vi "TMS Robot_adjust.vi"() -> ()   [LabVIEW 2018]
uses:
  <vilib>/Platform/TimedLoop/XDataNode/timing_clust.ctl
  <vilib>/Platform/TimedLoop/XDataNode/nitl_modes.ctl
  <vilib>/Platform/TimedLoop/XDataNode/wakeup.ctl
  <vilib>/myRIO/Instrument Drivers/Onboard IO/AI/typedefs/AI Reference.ctl
  <vilib>/myRIO/Common/Instrument Driver Framework/Utilities/typedefs/myRIO Generic Hardware Reference.ctl
  <vilib>/myRIO/Common/Instrument Driver Framework/Utilities/typedefs/Hardware Version Enum.ctl
  <vilib>/myRIO/Common/Instrument Driver Framework/Utilities/typedefs/myRIO v1.0 Reference.ctl
  <vilib>/myRIO/Common/Instrument Driver Framework/Utilities/typedefs/Generic FPGA Reference.ctl
  <vilib>/myRIO/Common/Instrument Driver Framework/myRIO v1.0/AI/typedefs/AI Channels List.ctl
  <vilib>/myRIO/Common/Instrument Driver Framework/myRIO v1.0/AI/typedefs/AI Channels Enum.ctl
  <vilib>/myRIO/Common/Instrument Driver Framework/Utilities/typedefs/Analog Scaling Constants List.ctl
  <vilib>/myRIO/Common/Instrument Driver Framework/Utilities/typedefs/Analog Scaling Constants.ctl
  <vilib>/userdefined/High Color/nirio_resource_hc.ctl
  <vilib>/myRIO/Instrument Drivers/Onboard IO/DIO/typedefs/DIO Reference.ctl
  <vilib>/myRIO/Common/Instrument Driver Framework/myRIO v1.0/DIO/typedefs/DIO Channels List.ctl
  <vilib>/myRIO/Common/Instrument Driver Framework/myRIO v1.0/DIO/typedefs/DIO Channels Enum.ctl
  <vilib>/myRIO/Common/Instrument Driver Framework/myRIO v1.0/AI/vis/myRIO v1.1 Open AI.vi
  <vilib>/myRIO/Common/Instrument Driver Framework/myRIO v1.0/DIO/vis/myRIO v1.1 Open DIO.vi
  <vilib>/myRIO/Common/Instrument Driver Framework/Utilities/vis/Validate Channels.vi
  <vilib>/myRIO/Common/Instrument Driver Framework/myRIO v1.0/AI/vis/myRIO v1.0 Reserve AI.vi
  <vilib>/myRIO/Common/Instrument Driver Framework/myRIO v1.0/DIO/vis/myRIO v1.0 Reserve DIO.vi
  <vilib>/myRIO/Common/Instrument Driver Framework/myRIO v1.0/DIO/vis/myRIO v1.0 Close DIO.vi
  <vilib>/myRIO/Common/Instrument Driver Framework/myRIO v1.0/AI/vis/myRIO v1.0 Build MUX Configuration AI.vi
  <vilib>/myRIO/Common/Instrument Driver Framework/myRIO v1.0/Resource Manager/vis/myRIO v1.0 Reserve Channel List.vi
  <vilib>/myRIO/Common/Instrument Driver Framework/myRIO v1.0/DIO/vis/myRIO v1.0 Build MUX Configuration DIO.vi
  <vilib>/myRIO/Common/Instrument Driver Framework/myRIO v1.0/DIO/vis/myRIO v1.0 Unreserve DIO.vi
  <vilib>/myRIO/Common/Instrument Driver Framework/myRIO v1.0/Resource Manager/vis/myRIO v1.0 Reserve Channel.vi
  <vilib>/myRIO/Common/Instrument Driver Framework/myRIO v1.0/Resource Manager/vis/myRIO v1.0 Unreserve Channel.vi
  <vilib>/myRIO/Common/Instrument Driver Framework/myRIO v1.0/Resource Manager/vis/myRIO v1.0 Create Configuration List.vi
  <vilib>/myRIO/Common/Instrument Driver Framework/myRIO v1.0/Resource Manager/vis/myRIO v1.0 Unreserve Channel List.vi
  <vilib>/myRIO/Common/Instrument Driver Framework/myRIO v1.0/Resource Manager/vis/myRIO v1.0 Build Mutex Name.vi
  <vilib>/Utility/VariantDataType/GetNumericInfo.vi
  <vilib>/Utility/error.llb/Error Cluster From Error Code.vi
  <vilib>/myRIO/Common/Instrument Driver Framework/myRIO v1.0/myRIO v1.1 Open.vi
  <vilib>/myRIO/Common/Instrument Driver Framework/Utilities/vis/IO Manager.vi
  <vilib>/myRIO/Common/Instrument Driver Framework/Utilities/vis/Configuration Manager.vi
  <vilib>/myRIO/Common/Instrument Driver Framework/myRIO v1.0/Resource Manager/vis/myRIO v1.0 Configure IO.vi
  <vilib>/myRIO/Common/Instrument Driver Framework/myRIO v1.0/myRIO v1.0 Close.vi
  <vilib>/myRIO/Common/Instrument Driver Framework/myRIO v1.0/AI/vis/myRIO v1.0 Get Scaling Constants AI.vi
  <vilib>/myRIO/Common/Instrument Driver Framework/myRIO v1.0/AI/vis/myRIO v1.0 Read AI.vi
  <vilib>/myRIO/Common/Instrument Driver Framework/myRIO v1.0/DIO/vis/myRIO v1.0 Write DIO.vi
  <vilib>/myRIO/Common/Instrument Driver Framework/myRIO v1.0/DIO/vis/myRIO v1.0 Shutdown DIO.vi
  <vilib>/platform/TimedLoop/XDataNode/XDataNode.xnode
  <vilib>/myRIO/Instrument Drivers/Onboard IO/DIO/vis/myRIO DIO Open.xnode
  <vilib>/myRIO/Instrument Drivers/Onboard IO/AI/vis/myRIO AI Open.xnode
  <vilib>/Platform/TimedLoop/XDataNode/XDNodeRunTimeDep.lvlib
  <vilib>/myRIO/Instrument Drivers/Onboard IO/DIO/DIO.lvlib
  <vilib>/myRIO/Instrument Drivers/Onboard IO/AI/AI.lvlib
panel:
  out "Optical R":dbl
  out "Optical L":dbl
  out "Optical psi":dbl
  out "Optical Z":dbl
  out "Optical Y":dbl
  out "Optical X":dbl
  in  "Stop number L":dbl
  in  "Stop number R":dbl
  in  "Stop number x":dbl
  in  "Stop number y":dbl
  in  "Stop number z":dbl
  in  "Stop number psi":dbl
  out "up L":bool
  out "left L":bool
  in  "Step/s  curve":dbl=4.0
  in  "Step difference L":dbl
  in  "Tab Control":enum32{"Azimuth", "Elevation"}(tab)
  in  "Right":bool
  in  "Left":bool
  out "Real Output theta":dbl
  in  "User Input theta":dbl
  in  "Up":bool
  in  "Down":bool
  out "Real Output Phi":dbl
  in  "User Input Phi":dbl=10.45218049
  in  "Motor Input L":dbl
  out "down L":bool
  out "right L":bool
  out "Moving":bool
  out "up R":bool
  out "left R":bool
  in  "Step difference R":dbl
  in  "Motor Input R":dbl
  out "down R":bool
  out "right R":bool
  out "Moving R":bool
  out "up z":bool
  out "down z":bool
  out "right z":bool
  out "left z":bool
  in  "Step/s z":dbl=4.0
  out "Motor Position z":dbl
  in  "User Input z":dbl
  out "Motor State z":dbl
  out "Real Output z":dbl
  in  "Step diff z":dbl
  in  "Up z":bool
  in  "Motor Input z":dbl
  in  "Down z":bool
  out "Moving z":bool
  out "up x":bool
  out "down x":bool
  out "right x":bool
  out "left x":bool
  in  "Step/s x":dbl=4.0
  out "Motor Position x":dbl
  in  "User Input x":dbl
  out "Motor State x":dbl
  out "Real Output x":dbl
  in  "Step diff x":dbl
  in  "Forward x":bool
  in  "Motor Input x":dbl
  in  "Backward x":bool
  out "Moving x":bool
  out "up y":bool
  out "down y":bool
  out "right y":bool
  out "left y":bool
  in  "Step/s y":dbl=4.0
  out "Motor Position y":dbl
  in  "User Input y":dbl
  out "Motor State y":dbl
  out "Real Output y":dbl
  in  "Step diff y":dbl
  in  "Left y":bool
  in  "Motor Input y":dbl
  in  "Right y":bool
  out "Moving y":bool
  out "up psi":bool
  out "down psi":bool
  out "right psi":bool
  out "left psi":bool
  in  "Step/s psi":dbl=4.0
  out "Motor Position psi":dbl
  in  "User Input psi":dbl
  out "Motor State psi":dbl
  out "Real Output psi":dbl
  in  "Step diff psi":dbl
  in  "Left psi":bool
  in  "Motor Input psi":dbl
  in  "Right psi":bool
  out "Moving psi":bool
  in  "Stop":bool
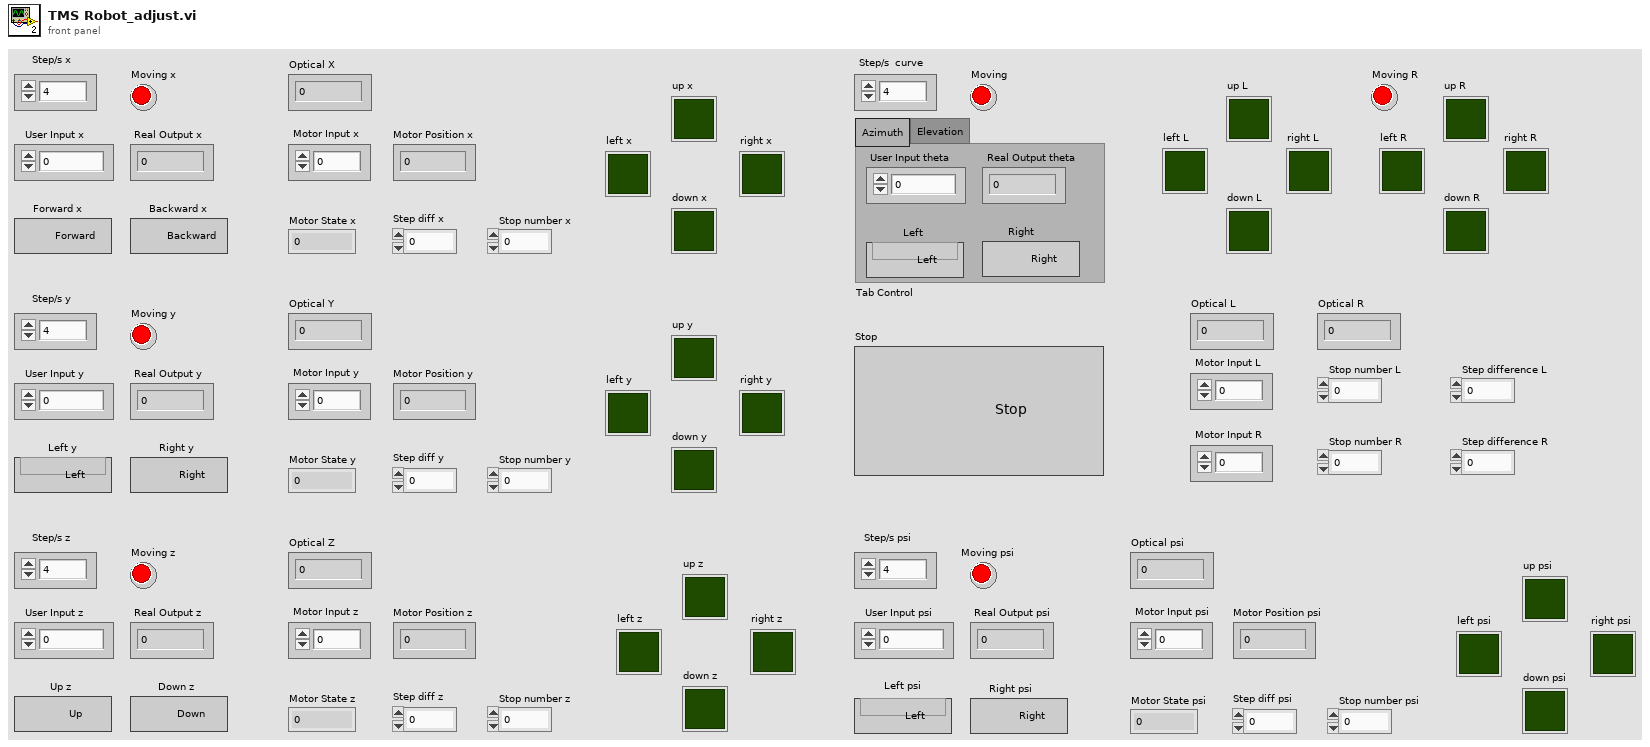
[diagram p1: front panel]
types:
  T1 = typedef "nirio_resource_hc.ctl" = tag
  T2 = typedef "Hardware Version Enum.ctl" = enum16{"Unknown", "myRIO-1900", "myRIO-1950", "roboRIO", "NI ELVIS RIO CM", "ELVIS III"}
  T3 = typedef "XDNodeRunTimeDep.lvlib/timing_clust.ctl" = cluster{"Expected End [f-1]":u64, "Actual End [f-1]":u64, "Finished Late? [f-1]":bool, "Expected End [i-1]":u64, "Actual End [i-1]":u64, "Finished Late? [i-1]":bool, "Expected Start [i]":u64, "Actual Start [i]":u64, "Expected Start [f]":u64, "Actual Start [f]":u64, "Source Name":string, "Structure Name":string, "Period":i64, "Deadline":i64, "Offset":i64, "Start":i64, "Priority":i32, "Timeout":i32, "Mode":T4, "Wakeup Reason":T5, "Error":errorcluster, "Source Type":string, "Secondary Source Type":string, "Global End Time":u64, "Global Start Time":u64, "Frame Duration":u64, "Iteration Duration":u64, "Assigned CPU":i32, "I/O Scan Engine Mode":u32}
  T4 = typedef "XDNodeRunTimeDep.lvlib/nitl_modes.ctl" = enum32{"No Change", "Process missed periods, maintain original phase", "Discard missed periods, maintain original phase", "Process missed periods, ignore original phase", "Discard missed periods, ignore original phase"}
  T5 = typedef "XDNodeRunTimeDep.lvlib/wakeup.ctl" = enum32{"Normal", "Aborted", "Asynchronous wakeup", "Timing source error", "Timed loop error", "Timeout"}
  T6 = typedef "AI.lvlib/AI Reference.ctl" = cluster{"myRIO Reference":T7, "AI Channels List":T10, "AI Scaling Constants List":T12}
  T7 = typedef "myRIO Generic Hardware Reference.ctl" = cluster{"myRIO Model":T2, "myRIO Hardware Reference":T8}
  T8 = typedef "myRIO v1.0 Reference.ctl" = cluster{"Generic FPGA Reference":T9, "Allow multiple opens":bool}
  T9 = typedef "Generic FPGA Reference.ctl" = refnum<k20>
  T10 = typedef "AI Channels List.ctl" = T11[]
  T11 = typedef "AI Channels Enum.ctl" = enum16{"Not Connected", "AudioIn/Left", "AudioIn/Right", "C/AI0", "C/AI1", "A/AI0", "A/AI1", "A/AI2", "A/AI3", "A/AI4", "A/AI5", "A/AI6", "A/AI7", "B/AI0", "B/AI1", "B/AI2", "B/AI3", "B/AI4", "B/AI5", "B/AI6", "B/AI7", "AI/AI0", "AI/AI1", "AI/AI2", "AI/AI3", "A/AI0 (DIFF)", "A/AI1 (DIFF)", "A/AI2 (DIFF)", "A/AI3 (DIFF)", "B/AI0 (DIFF)", "B/AI1 (DIFF)", "B/AI2 (DIFF)", "B/AI3 (DIFF)"}
  T12 = typedef "Analog Scaling Constants List.ctl" = T13[]
  T13 = typedef "Analog Scaling Constants.ctl" = cluster{"LSB Weight (Volts)":dbl, "Offset (Volts)":dbl, "Signed?":bool}
  T14 = typedef "DIO.lvlib/DIO Reference.ctl" = cluster{"myRIO Reference":T7, "DIO Channels List":T15}
  T15 = typedef "DIO Channels List.ctl" = T16[]
  T16 = typedef "DIO Channels Enum.ctl" = enum16{"Not Connected", "C/DIO0", "C/DIO1", "C/DIO2", "C/DIO3", "C/DIO4", "C/DIO5", "C/DIO6", "C/DIO7", "A/DIO0", "A/DIO1", "A/DIO2", "A/DIO3", "A/DIO4", "A/DIO5", "A/DIO6", "A/DIO7", "A/DIO8", "A/DIO9", "A/DIO10", "A/DIO11", "A/DIO12", "A/DIO13", "A/DIO14", "A/DIO15", "A/DIO16", "A/DIO17", "A/DIO18", "A/DIO19", "B/DIO0", "B/DIO1", "B/DIO2", "B/DIO3", "B/DIO4", "B/DIO5", "B/DIO6", "B/DIO7", "B/DIO8", "B/DIO9", "B/DIO10", "B/DIO11", "B/DIO12", "B/DIO13", "B/DIO14", "B/DIO15", "B/DIO16", "B/DIO17", "B/DIO18", "B/DIO19", "LED0", "LED1", "LED2", "LED3", "Button0", "DIO/DIO0", "DIO/DIO1", "DIO/DIO2", "DIO/DIO3", "DIO/DIO4", "DIO/DIO5", "DIO/DIO6", "DIO/DIO7", "DIO/DIO8", "DIO/DIO9", "SPI/CS0", "SPI/CS1", "SPI/CS2", "SPI/CS3", "LED RADIO (Green)", "LED RADIO (Red)", "LED COMM (Green)", "LED COMM (Red)", "LED MODE (Green)", "LED MODE (Red)"}
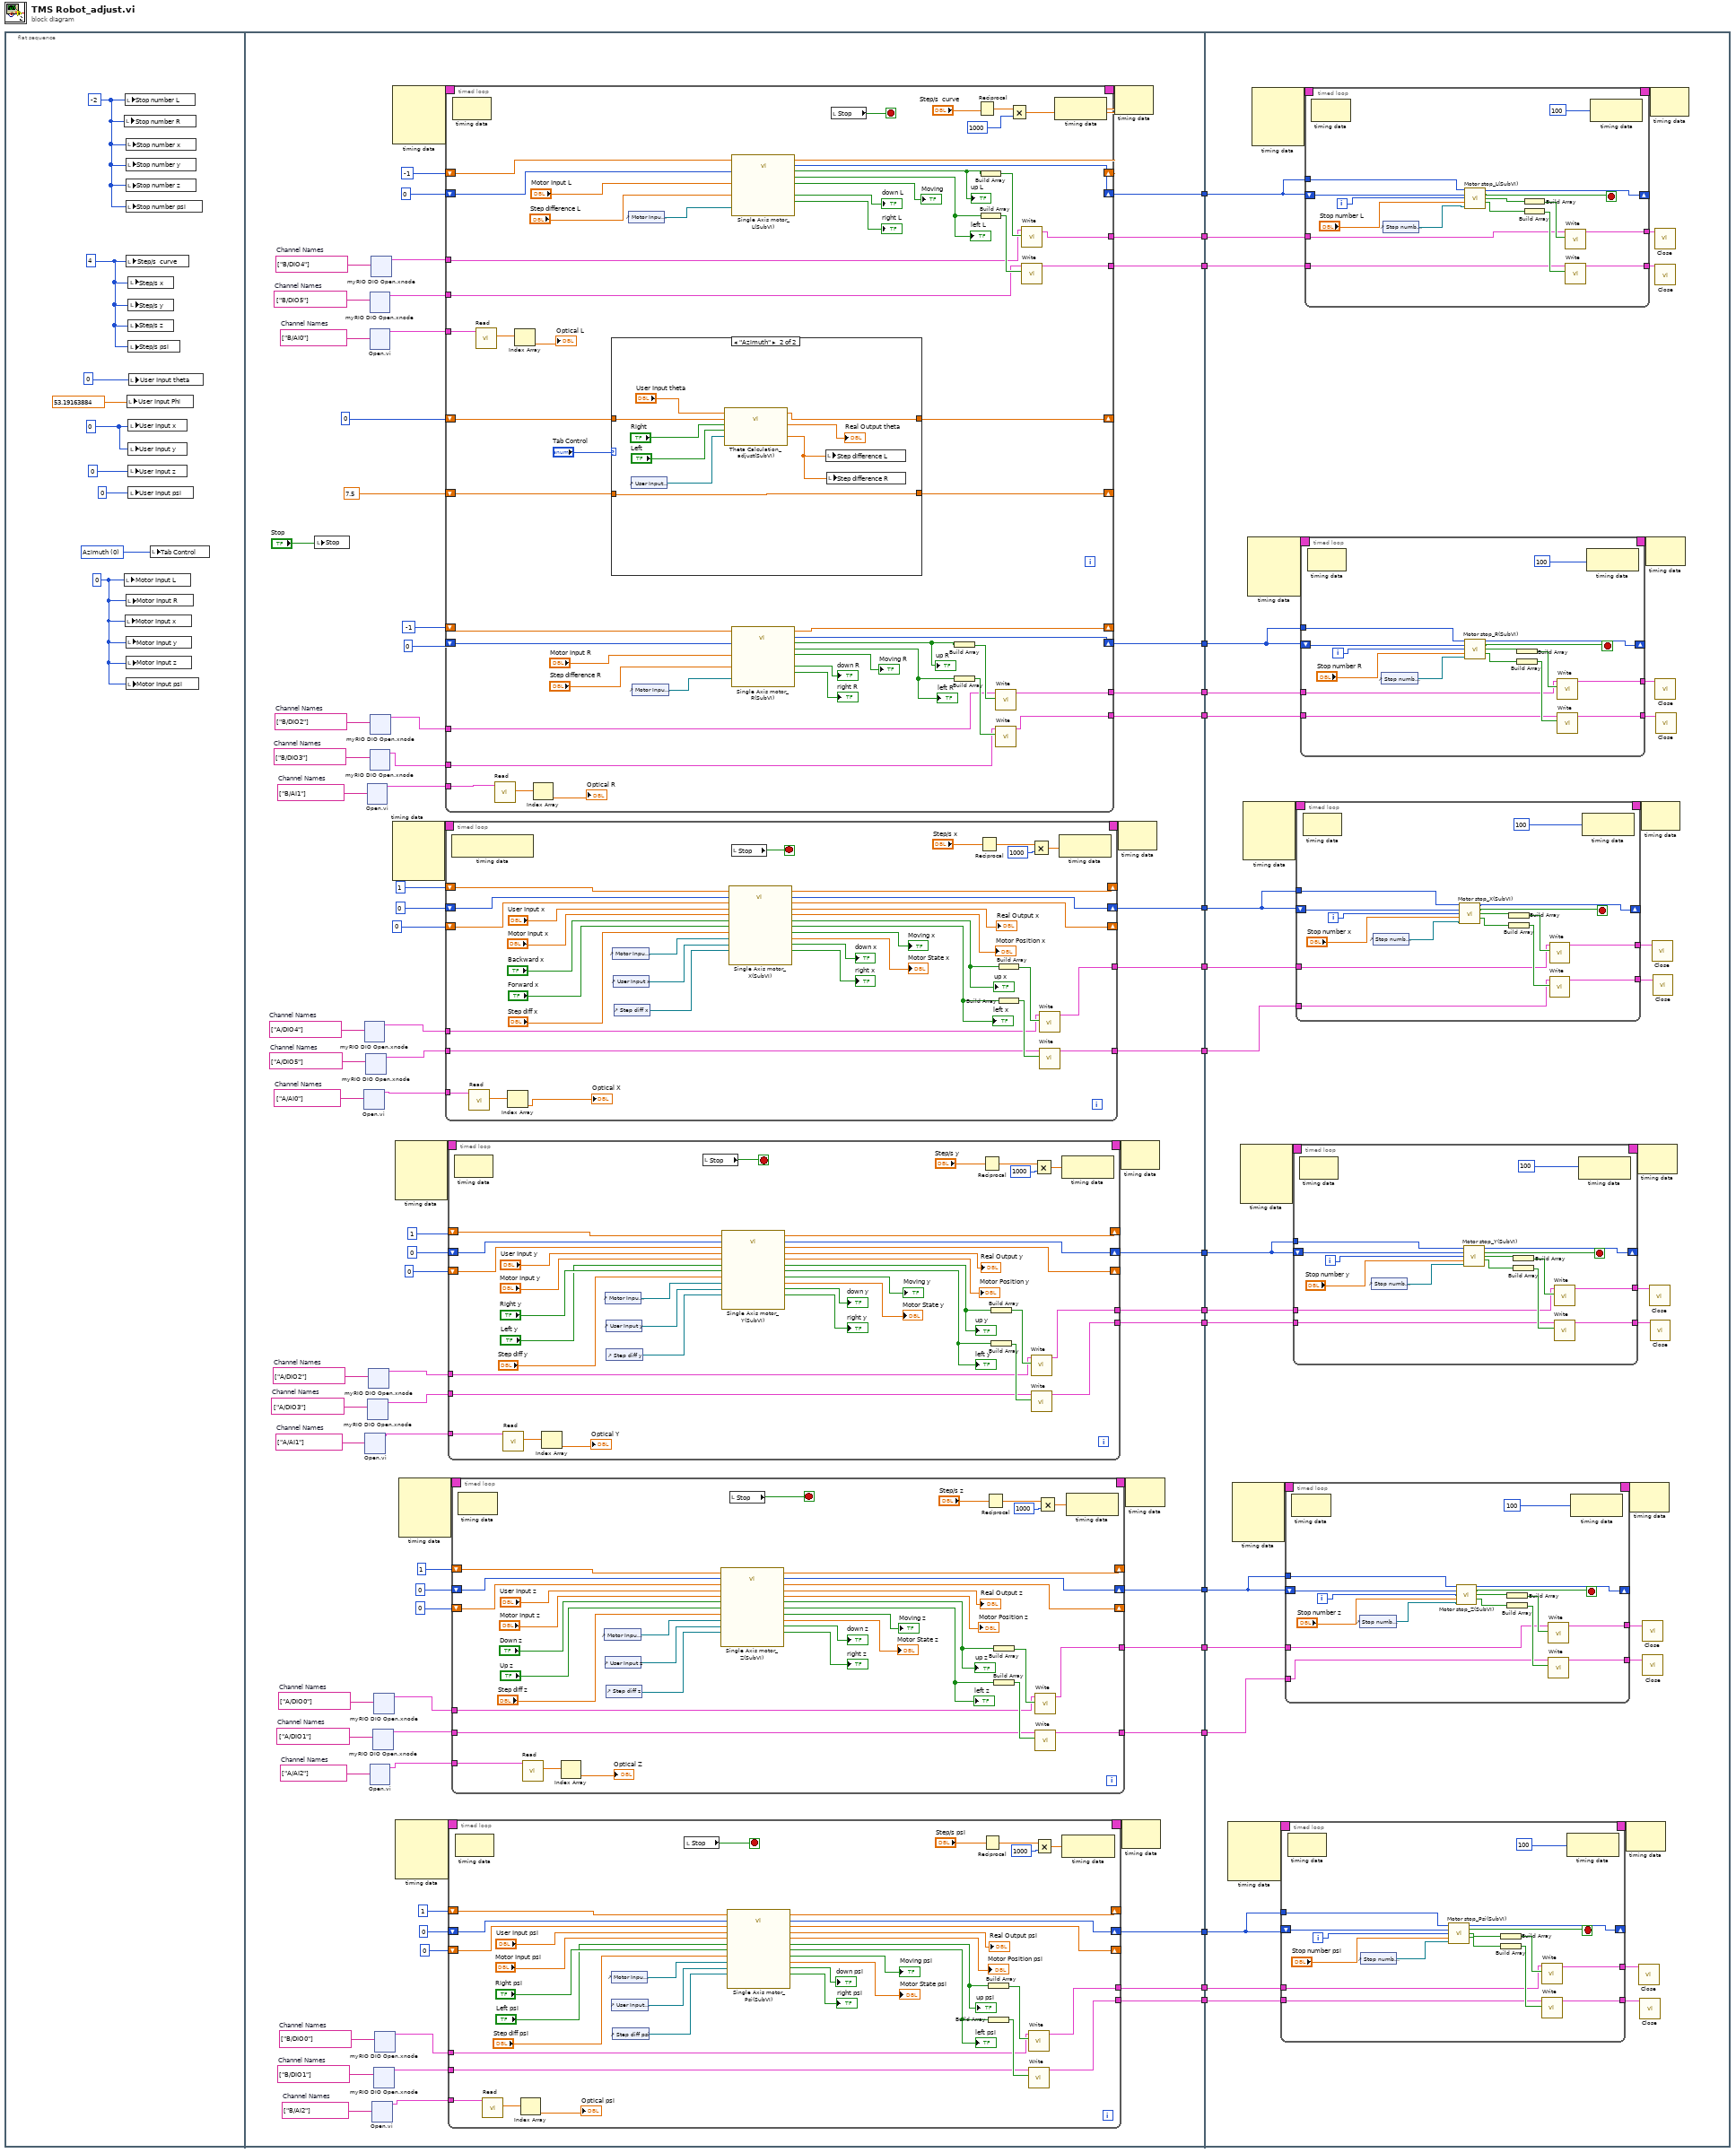
[diagram p0: block diagram]
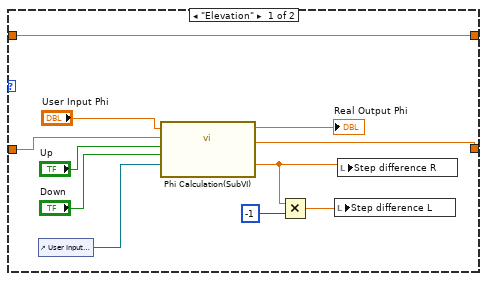
[diagram p2: hidden frame]
diagram:
  n1 = flat-sequence {
    tunnel: [w88] -> w18
    tunnel: [w87] -> w17
    tunnel: [w86] -> w16
    tunnel: [w85] -> w15
    tunnel: [w84] -> w14
    tunnel: [w83] -> w13
    tunnel: [w82] -> w12
    tunnel: [w81] -> w11
    tunnel: [w80] -> w10
    tunnel: [w79] -> w9
    tunnel: [w78] -> w8
    tunnel: [w77] -> w7
    tunnel: [w76] -> w6
    tunnel: [w75] -> w5
    tunnel: [w74] -> w4
    tunnel: [w73] -> w3
    tunnel: [w72] -> w2
    tunnel: [w71] -> w1
    tunnel: w18 -> [w696]
    tunnel: w17 -> [w693]
    tunnel: w16 -> [w690]
    tunnel: w15 -> [w687]
    tunnel: w14 -> [w684]
    tunnel: w13 -> [w681]
    tunnel: w12 -> [w678]
    tunnel: w11 -> [w677]
    tunnel: w10 -> [w676]
    tunnel: w9 -> [w675]
    tunnel: w8 -> [w670]
    tunnel: w7 -> [w669]
    tunnel: w6 -> [w668]
    tunnel: w5 -> [w667]
    tunnel: w4 -> [w666]
    tunnel: w3 -> [w665]
    tunnel: w2 -> [w664]
    tunnel: w1 -> [w663]
    frame #0 {
      w19 = 0
      w20 = u16 0 items=["Azimuth"]
      w22 = 0
      w26 = -2
      w25 = 4
      n2 = local write "Stop number R"(w26) -> ()
      n3 = local write "Motor Input L"(w19) -> ()
      n4 = local write "Stop number L"(w26) -> ()
      n5 = local write "Motor Input x"(w19) -> ()
      n6 = local write "Stop number x"(w26) -> ()
      n7 = local write "Stop number y"(w26) -> ()
      n8 = local write "Stop number z"(w26) -> ()
      n9 = local write "Stop number psi"(w26) -> ()
      n10 = local write "Motor Input R"(w19) -> ()
      n11 = local write "Motor Input y"(w19) -> ()
      n12 = local write "Motor Input z"(w19) -> ()
      n13 = local write "Motor Input psi"(w19) -> ()
      n14 = local write "Step/s  curve"(w25) -> ()
      n15 = local write "User Input Phi"(53.19163884) -> ()
      n16 = local write "Step/s x"(w25) -> ()
      n17 = local write "Step/s y"(w25) -> ()
      n18 = local write "Step/s z"(w25) -> ()
      n19 = local write "Step/s psi"(w25) -> ()
      n20 = local write "User Input x"(w22) -> ()
      n21 = local write "User Input y"(w22) -> ()
      n22 = local write "User Input z"(0) -> ()
      n23 = local write "User Input psi"(0) -> ()
      n24 = local write "User Input theta"(0) -> ()
      n25 = local write "Tab Control"(w20) -> ()
    }
    frame #1 {
      w36 = tag[] ["B/AI0"]  # Channel Names
      w38 = tag[] ["B/AI1"]  # Channel Names
      w41 = tag[] ["B/AI2"]  # Channel Names
      w43 = tag[] ["A/AI2"]  # Channel Names
      w45 = tag[] ["A/AI1"]  # Channel Names
      w47 = tag[] ["A/AI0"]  # Channel Names
      w51 = tag[] ["B/DIO1"]  # Channel Names
      w50 = tag[] ["B/DIO0"]  # Channel Names
      w55 = tag[] ["A/DIO1"]  # Channel Names
      w54 = tag[] ["A/DIO0"]  # Channel Names
      w59 = tag[] ["A/DIO3"]  # Channel Names
      w58 = tag[] ["A/DIO2"]  # Channel Names
      w63 = tag[] ["A/DIO5"]  # Channel Names
      w62 = tag[] ["A/DIO4"]  # Channel Names
      w67 = tag[] ["B/DIO5"]  # Channel Names
      w66 = tag[] ["B/DIO4"]  # Channel Names
      w70 = tag[] ["B/DIO3"]  # Channel Names
      w69 = tag[] ["B/DIO2"]  # Channel Names
      n26 = local write "Stop"("Stop") -> ()
      n27 = xnode "Open.vi"("Channel Names"=w47) -> ("AI Ref Out"=w46:T6)  [unwired: 2 in, 1 out]
      n28 = xnode "myRIO DIO Open.xnode"("Channel Names"=w62) -> ("DIO Ref Out"=w61:T14)  [unwired: 2 in, 1 out]
      n29 = xnode "Open.vi"("Channel Names"=w45) -> ("AI Ref Out"=w44:T6)  [unwired: 2 in, 1 out]
      n30 = xnode "myRIO DIO Open.xnode"("Channel Names"=w63) -> ("DIO Ref Out"=w60:T14)  [unwired: 2 in, 1 out]
      n31 = xnode "Open.vi"("Channel Names"=w38) -> ("AI Ref Out"=w37:T6)  [unwired: 2 in, 1 out]
      n32 = xnode "myRIO DIO Open.xnode"("Channel Names"=w59) -> ("DIO Ref Out"=w56:T14)  [unwired: 2 in, 1 out]
      n33 = xnode "myRIO DIO Open.xnode"("Channel Names"=w58) -> ("DIO Ref Out"=w57:T14)  [unwired: 2 in, 1 out]
      n34 = xnode "myRIO DIO Open.xnode"("Channel Names"=w67) -> ("DIO Ref Out"=w64:T14)  [unwired: 2 in, 1 out]
      n35 = xnode "Open.vi"("Channel Names"=w36) -> ("AI Ref Out"=w35:T6)  [unwired: 2 in, 1 out]
      n36 = xnode "myRIO DIO Open.xnode"("Channel Names"=w70) -> ("DIO Ref Out"=w39:T14)  [unwired: 2 in, 1 out]
      n37 = xnode "Open.vi"("Channel Names"=w43) -> ("AI Ref Out"=w42:T6)  [unwired: 2 in, 1 out]
      n38 = xnode "myRIO DIO Open.xnode"("Channel Names"=w69) -> ("DIO Ref Out"=w68:T14)  [unwired: 2 in, 1 out]
      n39 = xnode "myRIO DIO Open.xnode"("Channel Names"=w66) -> ("DIO Ref Out"=w65:T14)  [unwired: 2 in, 1 out]
      n40 = xnode "Open.vi"("Channel Names"=w41) -> ("AI Ref Out"=w40:T6)  [unwired: 2 in, 1 out]
      n41 = xnode "myRIO DIO Open.xnode"("Channel Names"=w55) -> ("DIO Ref Out"=w52:T14)  [unwired: 2 in, 1 out]
      n42 = xnode "myRIO DIO Open.xnode"("Channel Names"=w54) -> ("DIO Ref Out"=w53:T14)  [unwired: 2 in, 1 out]
      n43 = xnode "myRIO DIO Open.xnode"("Channel Names"=w51) -> ("DIO Ref Out"=w48:T14)  [unwired: 2 in, 1 out]
      n44 = xnode "myRIO DIO Open.xnode"("Channel Names"=w50) -> ("DIO Ref Out"=w49:T14)  [unwired: 2 in, 1 out]
      n45 = node-c288() -> (w103:T3)  [unwired: 4 in]
      n46 = node-c288() -> (w110:T3)  [unwired: 4 in]
      n47 = node-c288() -> (w101:T3)  [unwired: 4 in]
      n48 = node-c288() -> (w93:T3)  [unwired: 4 in]
      n49 = node-c288() -> (w105:T3)  [unwired: 4 in]
      n50 = timed-loop {
        shift-right: [w514] -> w86
        shift-left: 0 -> [w525]
        shift-right: [w515] -> _
        shift-left: 1 -> [w526]
        shift-right: [w510] -> _
        shift-left: 0 -> [w524]
        timing: w103 -> [_]
        timing-out: [_] -> w102
        tunnel: w61 -> [w501]
        tunnel: w60 -> [w500]
        tunnel: [w499] -> w78
        tunnel: [w498] -> w77
        tunnel: w46 -> [w496]
        stop <- w508 stop-if-true
        n51 = node-c288() -> ()  [unwired: 1 in, 1 out]
        n52 = call <vilib>:"Read.vi"("AI Ref In"=w496) -> ("Values"=w497:dbl[])  [unwired: 8 in, 2 out]
        n53 = Index Array(array=w497) -> (element=→"Optical X":dbl)  [unwired: 1 in]
        n54 = control-ref of="Motor Input x"() -> (w518:refnum<vi>)
        n55 = control-ref of="User Input x"() -> (w517:refnum<vi>)
        n56 = control-ref of="Step diff x"() -> (w516:refnum<vi>)
        n57 = call "Single Axis motor_X(SubVI).vi"("State=1, I"=w526, "Motor=0, I"=w525, "Position=0, I"=w524, "User Input"="User Input x", "Motor Input"="Motor Input x", "Backward"="Backward x", "Forward"="Forward x", "Step diff"="Step diff x", "Motor input_L"=w518, "User input_L"=w517, "Step diff_L"=w516) -> ("right"=→"right x":bool, "down"=→"down x":bool, "Motor State"=→"Motor State x":dbl, "State=1, O"=w515:dbl, "Motor=0, O"=w514:i32, "Position=0, O"=w510:dbl, "Real Output"=→"Real Output x":dbl, "Motor Position"=→"Motor Position x":dbl, "up"=w503:bool, "left"=w502:bool, "Moving"=→"Moving x":bool)  [unwired: 5 in, 1 out]
        "up x" <- w503
        "left x" <- w502
        n58 = local read "Stop"() -> (w508:bool)
        n59 = Reciprocal(x="Step/s x") -> (1/x=w529:dbl)
        n60 = Build Array(w503) -> (w505:bool[])
        n61 = Build Array(w502) -> (w504:bool[])
        n62 = Multiply(x=w529, y=1000) -> (x*y=w527:dbl)
        n63 = call <vilib>:"Write.vi"("Values"=w505, "DIO Ref In"=w501) -> ("DIO Ref Out"=w498:T14)  [unwired: 7 in, 1 out]
        n64 = call <vilib>:"Write.vi"("Values"=w504, "DIO Ref In"=w500) -> ("DIO Ref Out"=w499:T14)  [unwired: 7 in, 1 out]
        n65 = node-c288(w527) -> ()  [unwired: 1 out]
      }
      n66 = timed-loop {
        shift-right: [w618] -> w88
        shift-left: 0 -> [w619]
        shift-right: [w620] -> _
        shift-left: -1 -> [w621]
        shift-right: [w625] -> _
        shift-left: 0 -> [w626]
        timing: w110 -> [_]
        timing-out: [_] -> w109
        shift-right: [w623] -> _
        shift-left: 7.5 -> [w622]
        shift-right: [w607] -> w87
        shift-left: 0 -> [w608]
        shift-right: [w605] -> _
        shift-left: -1 -> [w606]
        tunnel: w68 -> [w596]
        tunnel: w39 -> [w595]
        tunnel: w64 -> [w590]
        tunnel: w65 -> [w589]
        tunnel: [w588] -> w82
        tunnel: [w587] -> w81
        tunnel: [w586] -> w80
        tunnel: [w585] -> w79
        tunnel: w37 -> [w583]
        tunnel: w35 -> [w581]
        stop <- w613 stop-if-true
        n67 = node-c288() -> ()  [unwired: 1 in, 1 out]
        n68 = call <vilib>:"Read.vi"("AI Ref In"=w581) -> ("Values"=w582:dbl[])  [unwired: 8 in, 2 out]
        n69 = call <vilib>:"Read.vi"("AI Ref In"=w583) -> ("Values"=w584:dbl[])  [unwired: 8 in, 2 out]
        n70 = Index Array(array=w582) -> (element=→"Optical L":dbl)  [unwired: 1 in]
        n71 = Index Array(array=w584) -> (element=→"Optical R":dbl)  [unwired: 1 in]
        n72 = case shown="\"Azimuth\"" "Tab Control" {
          tunnel: w622 -> [w640 w650]
          tunnel: [w639 w650] -> w623
          tunnel: w626 -> [w641 w647]
          tunnel: [w641 w646] -> w625
          frame "Elevation" {
            n73 = control-ref of="User Input Phi"() -> (w634:refnum<vi>)
            n74 = call "Phi Calculation(SubVI).vi"(0:"User Input Phi"="User Input Phi", "Position=0, I"=w640, "Up"="Up", "Down"="Down", 11:"User Input Phi"=w634) -> ("Real output phi"=→"Real Output Phi":dbl, "Position=0, O"=w639:dbl, "Step diff"=w631:dbl)  [unwired: 8 in]
            n75 = Multiply(x=w631, y=-1) -> (x*y=w632:dbl)
            n76 = local write "Step difference L"(w632) -> ()
            n77 = local write "Step difference R"(w631) -> ()
          }
          frame "Azimuth" {
            n78 = control-ref of="User Input theta"() -> (w648:refnum<vi>)
            n79 = call "Theta Calculation_adjust(SubVI).vi"(0:"User Input theta"="User Input theta", "Position=-85, I"=w647, "Right"="Right", "Left"="Left", 11:"User Input theta"=w648) -> ("Position=-85, O"=w646:dbl, "Real output theta"=→"Real Output theta":dbl, "Step diff"=w644:dbl)  [unwired: 8 in]
            n80 = local write "Step difference L"(w644) -> ()
            n81 = local write "Step difference R"(w644) -> ()
          }
        }
        n82 = control-ref of="Motor Input L"() -> (w615:refnum<vi>)
        n83 = control-ref of="Motor Input R"() -> (w610:refnum<vi>)
        n84 = call "Single Axis motor_R(SubVI).vi"("State=1, I"=w606, "Motor=0, I"=w608, "Motor Input"="Motor Input R", "Step diff"="Step difference R", "Motor Input_L"=w610) -> ("right"=→"right R":bool, "State=1, O"=w605:dbl, "Motor=0, O"=w607:i32, "up"=w598:bool, "left"=w597:bool, "Moving"=→"Moving R":bool, "down"=→"down R":bool)  [unwired: 14 in, 2 out]
        "up R" <- w598
        "left R" <- w597
        n85 = call "Single Axis motor_L(SubVI).vi"("State=1, I"=w621, "Motor=0, I"=w619, "Motor Input"="Motor Input L", "Step diff"="Step difference L", "Motor Input_L"=w615) -> ("right"=→"right L":bool, "State=1, O"=w620:dbl, "Motor=0, O"=w618:i32, "up"=w592:bool, "left"=w591:bool, "Moving"=→"Moving":bool, "down"=→"down L":bool)  [unwired: 14 in, 2 out]
        "up L" <- w592
        "left L" <- w591
        n86 = local read "Stop"() -> (w613:bool)
        n87 = Build Array(w598) -> (w600:bool[])
        n88 = Build Array(w597) -> (w599:bool[])
        n89 = Reciprocal(x="Step/s  curve") -> (1/x=w629:dbl)
        n90 = Build Array(w592) -> (w594:bool[])
        n91 = Build Array(w591) -> (w593:bool[])
        n92 = call <vilib>:"Write.vi"("Values"=w600, "DIO Ref In"=w596) -> ("DIO Ref Out"=w586:T14)  [unwired: 7 in, 1 out]
        n93 = call <vilib>:"Write.vi"("Values"=w599, "DIO Ref In"=w595) -> ("DIO Ref Out"=w585:T14)  [unwired: 7 in, 1 out]
        n94 = Multiply(x=w629, y=1000) -> (x*y=w627:dbl)
        n95 = call <vilib>:"Write.vi"("Values"=w594, "DIO Ref In"=w589) -> ("DIO Ref Out"=w588:T14)  [unwired: 7 in, 1 out]
        n96 = call <vilib>:"Write.vi"("Values"=w593, "DIO Ref In"=w590) -> ("DIO Ref Out"=w587:T14)  [unwired: 7 in, 1 out]
        n97 = node-c288(w627) -> ()  [unwired: 1 out]
      }
      n98 = timed-loop {
        shift-right: [w472] -> w85
        shift-left: 0 -> [w483]
        shift-right: [w473] -> _
        shift-left: 1 -> [w484]
        shift-right: [w469] -> _
        shift-left: 0 -> [w482]
        timing: w101 -> [_]
        timing-out: [_] -> w100
        tunnel: w57 -> [w459]
        tunnel: w56 -> [w458]
        tunnel: [w457] -> w76
        tunnel: [w456] -> w75
        tunnel: w44 -> [w454]
        stop <- w467 stop-if-true
        n99 = node-c288() -> ()  [unwired: 1 in, 1 out]
        n100 = call <vilib>:"Read.vi"("AI Ref In"=w454) -> ("Values"=w455:dbl[])  [unwired: 8 in, 2 out]
        n101 = Index Array(array=w455) -> (element=→"Optical Y":dbl)  [unwired: 1 in]
        n102 = control-ref of="Motor Input y"() -> (w476:refnum<vi>)
        n103 = control-ref of="User Input y"() -> (w475:refnum<vi>)
        n104 = control-ref of="Step diff y"() -> (w474:refnum<vi>)
        n105 = local read "Stop"() -> (w467:bool)
        n106 = call "Single Axis motor_Y(SubVI).vi"("State=1, I"=w484, "Motor=0, I"=w483, "Position=0, I"=w482, "User Input"="User Input y", "Motor Input"="Motor Input y", "Backward"="Left y", "Forward"="Right y", "Step diff"="Step diff y", "Motor input_L"=w476, "User input_L"=w475, "Step diff_L"=w474) -> ("right"=→"right y":bool, "down"=→"down y":bool, "Motor State"=→"Motor State y":dbl, "State=1, O"=w473:dbl, "Motor=0, O"=w472:i32, "Position=0, O"=w469:dbl, "Real Output"=→"Real Output y":dbl, "Motor Position"=→"Motor Position y":dbl, "up"=w461:bool, "left"=w460:bool, "Moving"=→"Moving y":bool)  [unwired: 5 in, 1 out]
        "up y" <- w461
        "left y" <- w460
        n107 = Reciprocal(x="Step/s y") -> (1/x=w487:dbl)
        n108 = Build Array(w461) -> (w463:bool[])
        n109 = Build Array(w460) -> (w462:bool[])
        n110 = call <vilib>:"Write.vi"("Values"=w463, "DIO Ref In"=w459) -> ("DIO Ref Out"=w456:T14)  [unwired: 7 in, 1 out]
        n111 = call <vilib>:"Write.vi"("Values"=w462, "DIO Ref In"=w458) -> ("DIO Ref Out"=w457:T14)  [unwired: 7 in, 1 out]
        n112 = Multiply(x=w487, y=1000) -> (x*y=w485:dbl)
        n113 = node-c288(w485) -> ()  [unwired: 1 out]
      }
      n114 = timed-loop {
        shift-right: [w430] -> w83
        shift-left: 0 -> [w441]
        shift-right: [w431] -> _
        shift-left: 1 -> [w442]
        shift-right: [w426] -> _
        shift-left: 0 -> [w440]
        timing: w93 -> [_]
        timing-out: [_] -> w92
        tunnel: w49 -> [w417]
        tunnel: w48 -> [w416]
        tunnel: [w415] -> w72
        tunnel: [w414] -> w71
        tunnel: w40 -> [w412]
        stop <- w424 stop-if-true
        n115 = node-c288() -> ()  [unwired: 1 in, 1 out]
        n116 = call <vilib>:"Read.vi"("AI Ref In"=w412) -> ("Values"=w413:dbl[])  [unwired: 8 in, 2 out]
        n117 = Index Array(array=w413) -> (element=→"Optical psi":dbl)  [unwired: 1 in]
        n118 = control-ref of="Motor Input psi"() -> (w434:refnum<vi>)
        n119 = control-ref of="User Input psi"() -> (w433:refnum<vi>)
        n120 = control-ref of="Step diff psi"() -> (w432:refnum<vi>)
        n121 = local read "Stop"() -> (w424:bool)
        n122 = call "Single Axis motor_Psi(SubVI).vi"("State=1, I"=w442, "Motor=0, I"=w441, "Position=0, I"=w440, "User Input"="User Input psi", "Motor Input"="Motor Input psi", "Backward"="Left psi", "Forward"="Right psi", "Step diff"="Step diff psi", "Motor input_L"=w434, "User input_L"=w433, "Step diff_L"=w432) -> ("right"=→"right psi":bool, "down"=→"down psi":bool, "Motor State"=→"Motor State psi":dbl, "State=1, O"=w431:dbl, "Motor=0, O"=w430:i32, "Position=0, O"=w426:dbl, "Real Output"=→"Real Output psi":dbl, "Motor Position"=→"Motor Position psi":dbl, "up"=w419:bool, "left"=w418:bool, "Moving"=→"Moving psi":bool)  [unwired: 5 in, 1 out]
        "up psi" <- w419
        "left psi" <- w418
        n123 = Reciprocal(x="Step/s psi") -> (1/x=w445:dbl)
        n124 = Build Array(w419) -> (w421:bool[])
        n125 = Build Array(w418) -> (w420:bool[])
        n126 = call <vilib>:"Write.vi"("Values"=w421, "DIO Ref In"=w417) -> ("DIO Ref Out"=w414:T14)  [unwired: 7 in, 1 out]
        n127 = call <vilib>:"Write.vi"("Values"=w420, "DIO Ref In"=w416) -> ("DIO Ref Out"=w415:T14)  [unwired: 7 in, 1 out]
        n128 = Multiply(x=w445, y=1000) -> (x*y=w443:dbl)
        n129 = node-c288(w443) -> ()  [unwired: 1 out]
      }
      n130 = timed-loop {
        shift-right: [w558] -> w84
        shift-left: 0 -> [w567]
        shift-right: [w559] -> _
        shift-left: 1 -> [w568]
        shift-right: [w554] -> _
        shift-left: 0 -> [w566]
        timing: w105 -> [_]
        timing-out: [_] -> w104
        tunnel: w53 -> [w543]
        tunnel: w52 -> [w542]
        tunnel: [w541] -> w74
        tunnel: [w540] -> w73
        tunnel: w42 -> [w538]
        stop <- w552 stop-if-true
        n131 = node-c288() -> ()  [unwired: 1 in, 1 out]
        n132 = call <vilib>:"Read.vi"("AI Ref In"=w538) -> ("Values"=w539:dbl[])  [unwired: 8 in, 2 out]
        n133 = Index Array(array=w539) -> (element=→"Optical Z":dbl)  [unwired: 1 in]
        n134 = control-ref of="Motor Input z"() -> (w562:refnum<vi>)
        n135 = control-ref of="User Input z"() -> (w561:refnum<vi>)
        n136 = control-ref of="Step diff z"() -> (w560:refnum<vi>)
        n137 = call "Single Axis motor_Z(SubVI).vi"("State=1, I"=w568, "Motor=0, I"=w567, "Position=0, I"=w566, "User Input"="User Input z", "Motor Input"="Motor Input z", "Backward"="Down z", "Forward"="Up z", "Step diff"="Step diff z", "Motor input_L"=w562, "User input_L"=w561, "Step diff_L"=w560) -> ("right"=→"right z":bool, "down"=→"down z":bool, "Motor State"=→"Motor State z":dbl, "State=1, O"=w559:dbl, "Motor=0, O"=w558:i32, "Position=0, O"=w554:dbl, "Real Output"=→"Real Output z":dbl, "Motor Position"=→"Motor Position z":dbl, "up"=w544:bool, "left"=w545:bool, "Moving"=→"Moving z":bool)  [unwired: 5 in, 1 out]
        "up z" <- w544
        "left z" <- w545
        n138 = local read "Stop"() -> (w552:bool)
        n139 = Reciprocal(x="Step/s z") -> (1/x=w571:dbl)
        n140 = Build Array(w544) -> (w547:bool[])
        n141 = Build Array(w545) -> (w546:bool[])
        n142 = call <vilib>:"Write.vi"("Values"=w547, "DIO Ref In"=w543) -> ("DIO Ref Out"=w540:T14)  [unwired: 7 in, 1 out]
        n143 = call <vilib>:"Write.vi"("Values"=w546, "DIO Ref In"=w542) -> ("DIO Ref Out"=w541:T14)  [unwired: 7 in, 1 out]
        n144 = Multiply(x=w571, y=1000) -> (x*y=w569:dbl)
        n145 = node-c288(w569) -> ()  [unwired: 1 out]
      }
      n146 = node-c288(w109) -> ()  [unwired: 1 out]
      n147 = node-c288(w102) -> ()  [unwired: 1 out]
      n148 = node-c288(w100) -> ()  [unwired: 1 out]
      n149 = node-c288(w92) -> ()  [unwired: 1 out]
      n150 = node-c288(w104) -> ()  [unwired: 1 out]
    }
    frame #2 {
      n151 = node-c288() -> (w683:T3)  [unwired: 4 in]
      n152 = node-c288() -> (w686:T3)  [unwired: 4 in]
      n153 = node-c288() -> (w689:T3)  [unwired: 4 in]
      n154 = node-c288() -> (w692:T3)  [unwired: 4 in]
      n155 = node-c288() -> (w695:T3)  [unwired: 4 in]
      n156 = node-c288() -> (w698:T3)  [unwired: 4 in]
      n157 = timed-loop {
        timing: w683 -> [_]
        timing-out: [_] -> w682
        shift-right: [w708] -> _
        shift-left: w681 -> [w712]
        tunnel: w681 -> [w713]
        tunnel: w664 -> [w702]
        tunnel: w663 -> [w701]
        tunnel: [w700] -> w658
        tunnel: [w699] -> w657
        i -> [w711]
        stop <- w707 stop-if-true
        n158 = node-c288() -> ()  [unwired: 1 in, 1 out]
        n159 = control-ref of="Stop number psi"() -> (w709:refnum<vi>)
        n160 = call "Motor stop_Psi(SubVI).vi"("Motor, C"=w713, "Motor, I"=w712, "i"=w711, "Stop number"="Stop number psi", "Stop number_L"=w709) -> ("Motor, O"=w708:i32, "Loop stop"=w707:bool, "up"=w704:bool, "left"=w703:bool)  [unwired: 7 in]
        n161 = Build Array(w704) -> (w705:bool[])
        n162 = Build Array(w703) -> (w706:bool[])
        n163 = call <vilib>:"Write.vi"("Values"=w705, "DIO Ref In"=w701) -> ("DIO Ref Out"=w700:T14)  [unwired: 7 in, 1 out]
        n164 = call <vilib>:"Write.vi"("Values"=w706, "DIO Ref In"=w702) -> ("DIO Ref Out"=w699:T14)  [unwired: 7 in, 1 out]
        n165 = node-c288(100) -> ()  [unwired: 1 out]
      }
      n166 = timed-loop {
        timing: w686 -> [_]
        timing-out: [_] -> w685
        shift-right: [w730] -> _
        shift-left: w684 -> [w734]
        tunnel: w684 -> [w735]
        tunnel: w666 -> [w723]
        tunnel: w665 -> [w724]
        tunnel: [w722] -> w660
        tunnel: [w721] -> w659
        i -> [w733]
        stop <- w729 stop-if-true
        n167 = node-c288() -> ()  [unwired: 1 in, 1 out]
        n168 = control-ref of="Stop number z"() -> (w731:refnum<vi>)
        n169 = call "Motor stop_Z(SubVI).vi"("Motor, C"=w735, "Motor, I"=w734, "i"=w733, "Stop number"="Stop number z", "Stop number_L"=w731) -> ("Motor, O"=w730:i32, "Loop stop"=w729:bool, "up"=w726:bool, "left"=w725:bool)  [unwired: 7 in]
        n170 = Build Array(w726) -> (w727:bool[])
        n171 = Build Array(w725) -> (w728:bool[])
        n172 = call <vilib>:"Write.vi"("Values"=w727, "DIO Ref In"=w724) -> ("DIO Ref Out"=w722:T14)  [unwired: 7 in, 1 out]
        n173 = call <vilib>:"Write.vi"("Values"=w728, "DIO Ref In"=w723) -> ("DIO Ref Out"=w721:T14)  [unwired: 7 in, 1 out]
        n174 = node-c288(100) -> ()  [unwired: 1 out]
      }
      n175 = timed-loop {
        timing: w689 -> [_]
        timing-out: [_] -> w688
        shift-right: [w752] -> _
        shift-left: w687 -> [w756]
        tunnel: w687 -> [w757]
        tunnel: w668 -> [w746]
        tunnel: w667 -> [w745]
        tunnel: [w744] -> w662
        tunnel: [w743] -> w661
        i -> [w755]
        stop <- w751 stop-if-true
        n176 = node-c288() -> ()  [unwired: 1 in, 1 out]
        n177 = control-ref of="Stop number y"() -> (w753:refnum<vi>)
        n178 = call "Motor stop_Y(SubVI).vi"("Motor, C"=w757, "Motor, I"=w756, "i"=w755, "Stop number"="Stop number y", "Stop number_L"=w753) -> ("Motor, O"=w752:i32, "Loop stop"=w751:bool, "up"=w748:bool, "left"=w747:bool)  [unwired: 7 in]
        n179 = Build Array(w748) -> (w749:bool[])
        n180 = Build Array(w747) -> (w750:bool[])
        n181 = call <vilib>:"Write.vi"("Values"=w749, "DIO Ref In"=w745) -> ("DIO Ref Out"=w744:T14)  [unwired: 7 in, 1 out]
        n182 = call <vilib>:"Write.vi"("Values"=w750, "DIO Ref In"=w746) -> ("DIO Ref Out"=w743:T14)  [unwired: 7 in, 1 out]
        n183 = node-c288(100) -> ()  [unwired: 1 out]
      }
      n184 = timed-loop {
        timing: w692 -> [_]
        timing-out: [_] -> w691
        shift-right: [w774] -> _
        shift-left: w690 -> [w778]
        tunnel: w690 -> [w779]
        tunnel: [w768] -> w672
        tunnel: [w767] -> w671
        tunnel: w670 -> [w766]
        tunnel: w669 -> [w765]
        i -> [w777]
        stop <- w773 stop-if-true
        n185 = node-c288() -> ()  [unwired: 1 in, 1 out]
        n186 = control-ref of="Stop number x"() -> (w775:refnum<vi>)
        n187 = call "Motor stop_X(SubVI).vi"("Motor, C"=w779, "Motor, I"=w778, "i"=w777, "Stop number"="Stop number x", "Stop number_L"=w775) -> ("Motor, O"=w774:i32, "Loop stop"=w773:bool, "up"=w770:bool, "left"=w769:bool)  [unwired: 7 in]
        n188 = Build Array(w770) -> (w771:bool[])
        n189 = Build Array(w769) -> (w772:bool[])
        n190 = call <vilib>:"Write.vi"("Values"=w771, "DIO Ref In"=w765) -> ("DIO Ref Out"=w768:T14)  [unwired: 7 in, 1 out]
        n191 = call <vilib>:"Write.vi"("Values"=w772, "DIO Ref In"=w766) -> ("DIO Ref Out"=w767:T14)  [unwired: 7 in, 1 out]
        n192 = node-c288(100) -> ()  [unwired: 1 out]
      }
      n193 = timed-loop {
        timing: w695 -> [_]
        timing-out: [_] -> w694
        shift-right: [w796] -> _
        shift-left: w693 -> [w800]
        tunnel: w693 -> [w801]
        tunnel: w676 -> [w790]
        tunnel: w675 -> [w789]
        tunnel: [w788] -> w674
        tunnel: [w787] -> w673
        i -> [w799]
        stop <- w795 stop-if-true
        n194 = node-c288() -> ()  [unwired: 1 in, 1 out]
        n195 = control-ref of="Stop number R"() -> (w797:refnum<vi>)
        n196 = call "Motor stop_R(SubVI).vi"("Motor, C"=w801, "Motor, I"=w800, "i"=w799, "Stop number"="Stop number R", "Stop number_L"=w797) -> ("Motor, O"=w796:i32, "Loop stop"=w795:bool, "up"=w792:bool, "left"=w791:bool)  [unwired: 7 in]
        n197 = Build Array(w792) -> (w793:bool[])
        n198 = Build Array(w791) -> (w794:bool[])
        n199 = call <vilib>:"Write.vi"("Values"=w793, "DIO Ref In"=w790) -> ("DIO Ref Out"=w788:T14)  [unwired: 7 in, 1 out]
        n200 = call <vilib>:"Write.vi"("Values"=w794, "DIO Ref In"=w789) -> ("DIO Ref Out"=w787:T14)  [unwired: 7 in, 1 out]
        n201 = node-c288(100) -> ()  [unwired: 1 out]
      }
      n202 = timed-loop {
        timing: w698 -> [_]
        timing-out: [_] -> w697
        shift-right: [w818] -> _
        shift-left: w696 -> [w822]
        tunnel: w696 -> [w823]
        tunnel: [w812] -> w680
        tunnel: [w811] -> w679
        tunnel: w678 -> [w810]
        tunnel: w677 -> [w809]
        i -> [w821]
        stop <- w817 stop-if-true
        n203 = node-c288() -> ()  [unwired: 1 in, 1 out]
        n204 = control-ref of="Stop number L"() -> (w819:refnum<vi>)
        n205 = call "Motor stop_L(SubVI).vi"("Motor, C"=w823, "Motor, I"=w822, "i"=w821, "Stop number"="Stop number L", "Stop number_L"=w819) -> ("Motor, O"=w818:i32, "Loop stop"=w817:bool, "up"=w814:bool, "left"=w813:bool)  [unwired: 7 in]
        n206 = Build Array(w814) -> (w815:bool[])
        n207 = Build Array(w813) -> (w816:bool[])
        n208 = call <vilib>:"Write.vi"("Values"=w815, "DIO Ref In"=w810) -> ("DIO Ref Out"=w812:T14)  [unwired: 7 in, 1 out]
        n209 = call <vilib>:"Write.vi"("Values"=w816, "DIO Ref In"=w809) -> ("DIO Ref Out"=w811:T14)  [unwired: 7 in, 1 out]
        n210 = node-c288(100) -> ()  [unwired: 1 out]
      }
      n211 = node-c288(w682) -> ()  [unwired: 1 out]
      n212 = node-c288(w685) -> ()  [unwired: 1 out]
      n213 = node-c288(w688) -> ()  [unwired: 1 out]
      n214 = call <vilib>:"Close.vi"("DIO Ref In"=w658) -> ()  [unwired: 10 in, 1 out]
      n215 = call <vilib>:"Close.vi"("DIO Ref In"=w657) -> ()  [unwired: 10 in, 1 out]
      n216 = node-c288(w691) -> ()  [unwired: 1 out]
      n217 = call <vilib>:"Close.vi"("DIO Ref In"=w660) -> ()  [unwired: 10 in, 1 out]
      n218 = call <vilib>:"Close.vi"("DIO Ref In"=w659) -> ()  [unwired: 10 in, 1 out]
      n219 = node-c288(w694) -> ()  [unwired: 1 out]
      n220 = call <vilib>:"Close.vi"("DIO Ref In"=w662) -> ()  [unwired: 10 in, 1 out]
      n221 = node-c288(w697) -> ()  [unwired: 1 out]
      n222 = call <vilib>:"Close.vi"("DIO Ref In"=w661) -> ()  [unwired: 10 in, 1 out]
      n223 = call <vilib>:"Close.vi"("DIO Ref In"=w672) -> ()  [unwired: 10 in, 1 out]
      n224 = call <vilib>:"Close.vi"("DIO Ref In"=w671) -> ()  [unwired: 10 in, 1 out]
      n225 = call <vilib>:"Close.vi"("DIO Ref In"=w680) -> ()  [unwired: 10 in, 1 out]
      n226 = call <vilib>:"Close.vi"("DIO Ref In"=w679) -> ()  [unwired: 10 in, 1 out]
      n227 = call <vilib>:"Close.vi"("DIO Ref In"=w674) -> ()  [unwired: 10 in, 1 out]
      n228 = call <vilib>:"Close.vi"("DIO Ref In"=w673) -> ()  [unwired: 10 in, 1 out]
    }
  }
